vi "PicoScope3000aAdvancedTriggerSettingsV2.vi"(0 "error in":errorcluster, 1 "handle in":i16, 3 "Trigger Conditions":T6 {"Condition Logic" items=["AND", "OR", "XOR"]}, 4 "Trigger Delay":u32, 5 "Auto Trigger (ms)":i32, 6 "Channel A Trigger Properties":T3 {"Direction" items=["Above / Inside", "Below / Outside", "Rising / Enter", "Falling / Exit", "Rising or Falling / Enter or Exit", "Above Lower", "Below Lower", "Rising Lower", "Falling Lower", "Positive Runt", "Negative Runt"]; "Threshold Mode" items=["Level", "Window"]}, 7 "Channel D Trigger Properties":T3 {"Direction" items=["Above / Inside", "Below / Outside", "Rising / Enter", "Falling / Exit", "Rising or Falling / Enter or Exit", "Above Lower", "Below Lower", "Rising Lower", "Falling Lower", "Positive Runt", "Negative Runt"]; "Threshold Mode" items=["Level", "Window"]}, 8 "Channel B Trigger Properties":T3 {"Direction" items=["Above / Inside", "Below / Outside", "Rising / Enter", "Falling / Exit", "Rising or Falling / Enter or Exit", "Above Lower", "Below Lower", "Rising Lower", "Falling Lower", "Positive Runt", "Negative Runt"]; "Threshold Mode" items=["Level", "Window"]}, 10 "Digital Port  0":T2 {"Direction Channel 7" items=["Don't Care", "Low", "High", "Rising", "Falling"]; "Direction Channel 6" items=["Don't Care", "Low", "High", "Rising", "Falling"]; "Direction Channel 5" items=["Don't Care", "Low", "High", "Rising", "Falling"]; "Direction Channel 4" items=["Don't Care", "Low", "High", "Rising", "Falling"]; "Direction Channel 3" items=["Don't Care", "Low", "High", "Rising", "Falling"]; "Direction Channel 2" items=["Don't Care", "Low", "High", "Rising", "Falling"]; "Direction Channel 1" items=["Don't Care", "Low", "High", "Rising", "Falling"]; "Direction Channel 0" items=["Don't Care", "Low", "High", "Rising", "Falling"]}, 11 "Ext. Trigger Properties":T3 {"Direction" items=["Above / Inside", "Below / Outside", "Rising / Enter", "Falling / Exit", "Rising or Falling / Enter or Exit", "Above Lower", "Below Lower", "Rising Lower", "Falling Lower", "Positive Runt", "Negative Runt"]; "Threshold Mode" items=["Level", "Window"]}, 12 "Digital Port  1":T1 {"Direction Channel 15" items=["Don't Care", "Low", "High", "Rising", "Falling"]; "Direction Channel 14" items=["Don't Care", "Low", "High", "Rising", "Falling"]; "Direction Channel 13" items=["Don't Care", "Low", "High", "Rising", "Falling"]; "Direction Channel 12" items=["Don't Care", "Low", "High", "Rising", "Falling"]; "Direction Channel 11" items=["Don't Care", "Low", "High", "Rising", "Falling"]; "Direction Channel 10" items=["Don't Care", "Low", "High", "Rising", "Falling"]; "Direction Channel 9" items=["Don't Care", "Low", "High", "Rising", "Falling"]; "Direction Channel 8" items=["Don't Care", "Low", "High", "Rising", "Falling"]}, 13 "Aux. Trigger Properties":T3 {"Direction" items=["Above / Inside", "Below / Outside", "Rising / Enter", "Falling / Exit", "Rising or Falling / Enter or Exit", "Above Lower", "Below Lower", "Rising Lower", "Falling Lower", "Positive Runt", "Negative Runt"]; "Threshold Mode" items=["Level", "Window"]}, 16 "Channel C Trigger Properties":T3 {"Direction" items=["Above / Inside", "Below / Outside", "Rising / Enter", "Falling / Exit", "Rising or Falling / Enter or Exit", "Above Lower", "Below Lower", "Rising Lower", "Falling Lower", "Positive Runt", "Negative Runt"]; "Threshold Mode" items=["Level", "Window"]}, 18 "Pulse Width Qualifier Conditions":T5 {"Condition Logic" items=["AND", "OR", "XOR"]}, 19 "Pulse Width Qualifier Settings":T4 {"Pulse Width Type" items=["None", "Less Than", "Greater Than", "In Range", "Out of Range"]; "Direction" items=["Rising", "Falling"]}) -> (14 "error out":errorcluster, 15 "handle out":i16)   [LabVIEW 2009]
doc: "This VI is an interface for the advanced trigger features of the oscilloscope (a simple trigger can be set using PicoScope3000aSettings.vi, in which case it is not necessary to use this VI)."
uses:
  ps3000a.dll
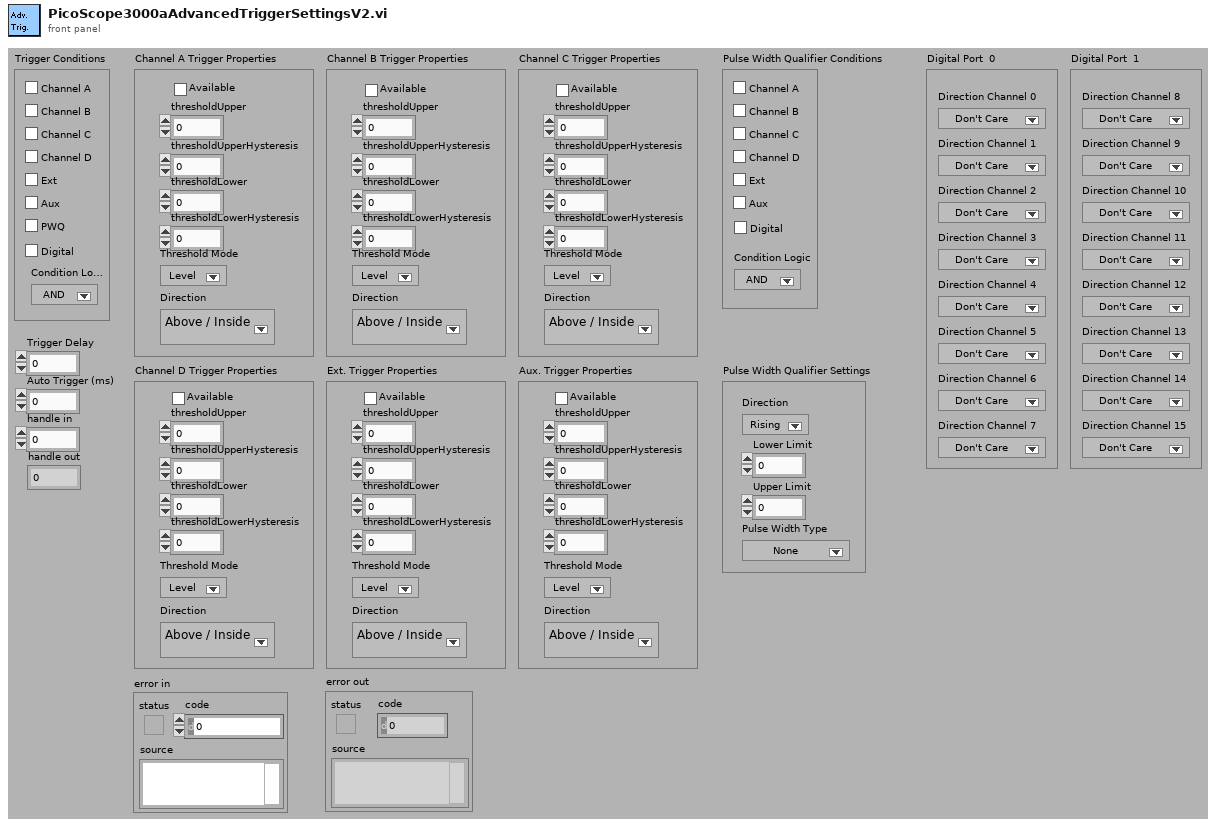
[diagram p1: front panel]
types:
  T1 = cluster{"Direction Channel 8":u16, "Direction Channel 9":u16, "Direction Channel 10":u16, "Direction Channel 11":u16, "Direction Channel 12":u16, "Direction Channel 13":u16, "Direction Channel 14":u16, "Direction Channel 15":u16}
  T2 = cluster{"Direction Channel 0":u16, "Direction Channel 1":u16, "Direction Channel 2":u16, "Direction Channel 3":u16, "Direction Channel 4":u16, "Direction Channel 5":u16, "Direction Channel 6":u16, "Direction Channel 7":u16}
  T3 = cluster{"thresholdUpper":i16, "thresholdUpperHysteresis":u16, "thresholdLower":i16, "thresholdLowerHysteresis":u16, "Threshold Mode":i32, "Direction":i32, "Available":bool}
  T4 = cluster{"Direction":u32, "Lower Limit":u32, "Upper Limit":u32, "Pulse Width Type":u32}
  T5 = cluster{"Channel A":bool, "Channel B":bool, "Channel C":bool, "Channel D":bool, "Aux":bool, "Condition Logic":u16, "Ext":bool, "Digital":bool}
  T6 = cluster{"Channel A":bool, "Channel B":bool, "Channel C":bool, "Channel D":bool, "Aux":bool, "PWQ":bool, "Condition Logic":u16, "Ext":bool, "Digital":bool}
  T7 = cluster{"thresholdUpper":i16, "thresholdUpperHysteresis":u16, "thresholdLower":i16, "thresholdLowerHysteresis":u16, "Threshold Mode":i32, "Direction":i32, "Available":bool}[]
  T8 = cluster{"[0]":u32, "[1]":u32, "[2]":u32, "[3]":u32, "[4]":u32, "[5]":u32, "[6]":u32, "[7]":u32, "[8]":u32}
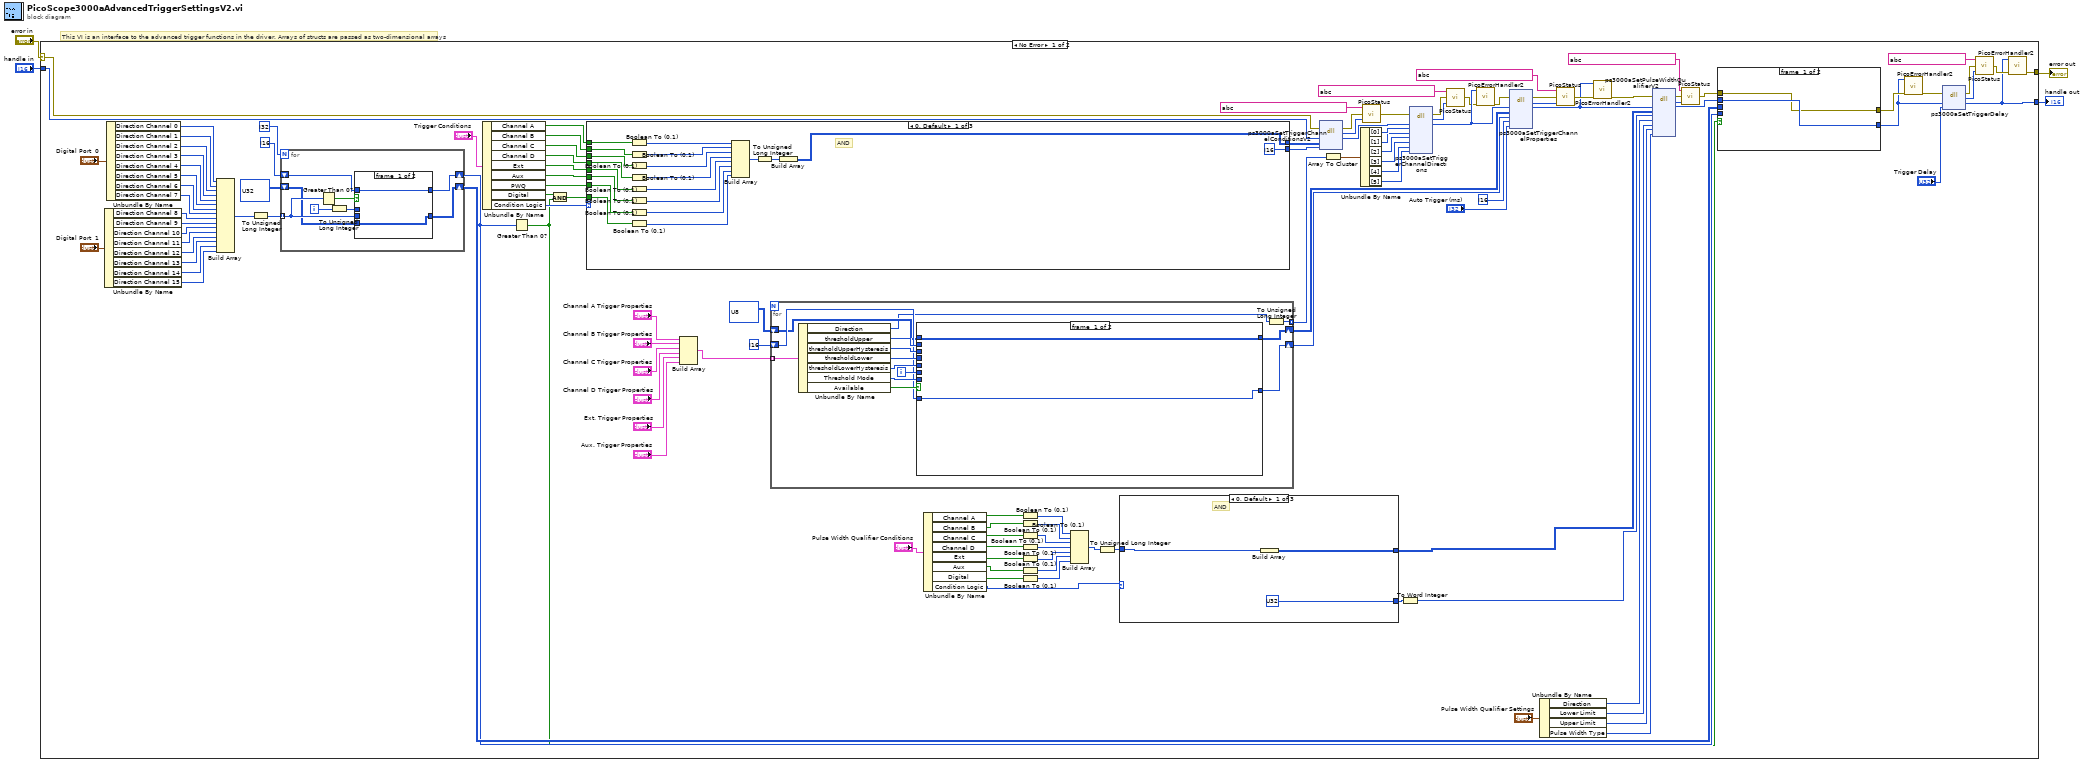
[diagram p0: block diagram]
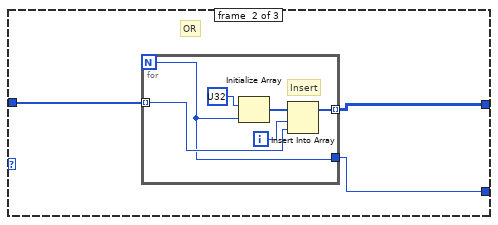
[diagram p2: hidden frame]
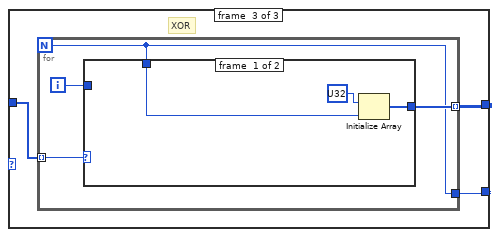
[diagram p3: hidden frame]
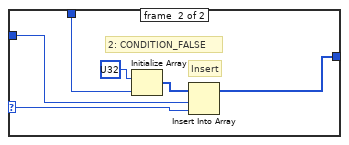
[diagram p4: hidden frame]
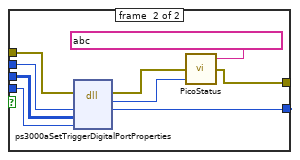
[diagram p5: hidden frame]
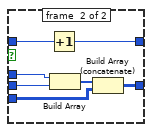
[diagram p6: hidden frame]
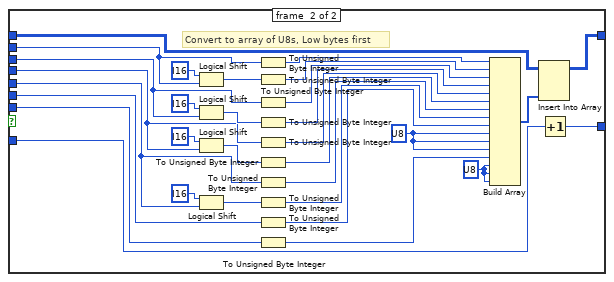
[diagram p7: hidden frame]
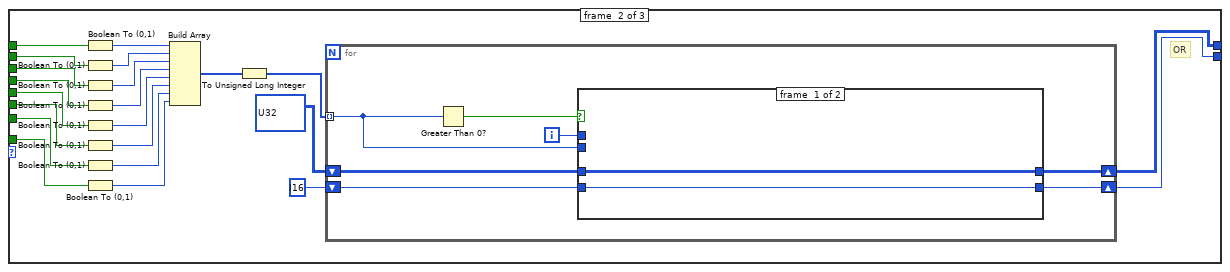
[diagram p8: hidden frame]
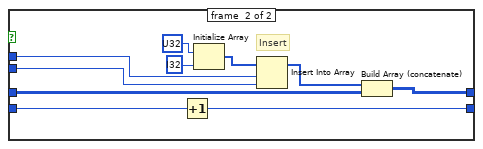
[diagram p9: hidden frame]
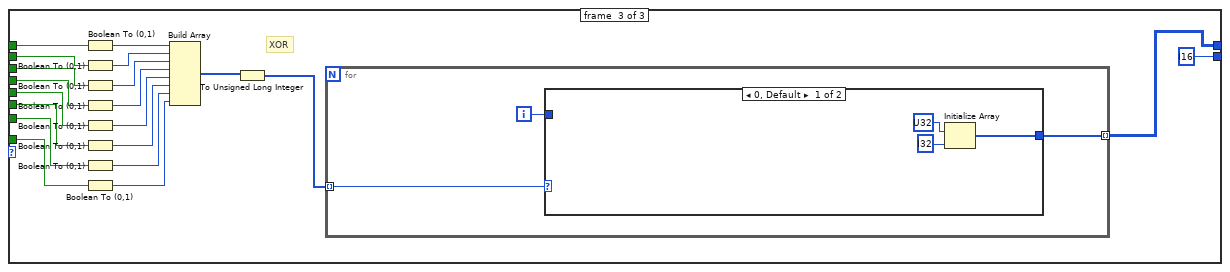
[diagram p10: hidden frame]
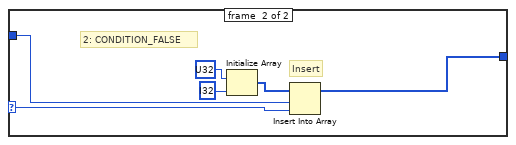
[diagram p11: hidden frame]
diagram:
  # "This VI is an interface to the advanced trigger functions in the driver. Arrays of structs are passed as two-dimensional arrays"
  n1 = case shown="No Error" "error in" {
    selector: "error in" -> [w93 w321]
    tunnel: "handle in" -> [w97 w322]
    tunnel: [w33 w322] -> w2
    tunnel: [w34 w321] -> w1
    frame #0 {
      n2 = Unbundle By Name("Digital Port  1") -> ("Direction Channel 8"=w58:u16, "Direction Channel 9"=w57:u16, "Direction Channel 10"=w56:u16, "Direction Channel 11"=w55:u16, "Direction Channel 12"=w54:u16, "Direction Channel 13"=w53:u16, "Direction Channel 14"=w52:u16, "Direction Channel 15"=w51:u16)
      n3 = Unbundle By Name("Digital Port  0") -> ("Direction Channel 0"=w70:u16, "Direction Channel 1"=w69:u16, "Direction Channel 2"=w68:u16, "Direction Channel 3"=w67:u16, "Direction Channel 4"=w66:u16, "Direction Channel 5"=w65:u16, "Direction Channel 6"=w64:u16, "Direction Channel 7"=w63:u16)
      n4 = Build Array(w70, w69, w68, w67, w66, w65, w64, w63, w58, w57, w56, w55, w54, w53, w52, w51) -> (w25:u16[])
      n5 = To Unsigned Long Integer(number=w25) -> (unsigned 32bit integer=w26:u32[])
      n6 = for {
        N: i32 ? -> [_]
        tunnel: w26 -> [w170] mode=indexing
        shift-right: [w169] -> w46
        shift-left: u32[][] ? -> [w168]
        shift-right: [w167] -> w43
        shift-left: i16 ? -> [w166]
        i -> [w164]
        n7 = Greater Than 0?(x=w170) -> (x > 0?=w171:bool)
        n8 = To Unsigned Long Integer(number=w164) -> (unsigned 32bit integer=w165:u32)
        n9 = case shown="True" w171 {
          tunnel: w165 -> [_ w180]
          tunnel: w170 -> [_ w179]
          tunnel: [w173 w177] -> w169
          tunnel: w168 -> [w173 w176]
          tunnel: [w172 w175] -> w167
          tunnel: w166 -> [w172 w174]
          frame #0 {
          }
          frame #1 {
            n10 = Increment(x=w174) -> (x+1=w175:i16)
            n11 = Build Array(w180, w179) -> (w178:u32[])
            n12 = Build Array (concatenate)(w178, w176) -> (w177:u32[][])
          }
        }
      }
      n13 = Unbundle By Name("Trigger Conditions") -> ("Channel A"=w77:bool, "Channel B"=w76:bool, "Channel C"=w75:bool, "Channel D"=w74:bool, "Ext"=w73:bool, "Aux"=w72:bool, "PWQ"=w71:bool, "Digital"=w45:bool, "Condition Logic"=w78:u16)
      n14 = Greater Than 0?(x=w43) -> (x > 0?=w42:bool)
      n15 = And(x=w45, y=w42) -> (x .and. y?=w44:bool)
      n16 = case shown="0, Default" w78 {
        tunnel: [w247 w262 w301] -> w121
        tunnel: [i16 ? w260 i16 ?] -> w120
        tunnel: w77 -> [w245 w257 w298]
        tunnel: w76 -> [w244 w256 w297]
        tunnel: w75 -> [w243 w255 w296]
        tunnel: w74 -> [w242 w254 w295]
        tunnel: w73 -> [w241 w253 w294]
        tunnel: w72 -> [w240 w252 w293]
        tunnel: w71 -> [w239 w251 w292]
        tunnel: w44 -> [w238 w250 w291]
        frame #0 {
          # "AND"
          n17 = Boolean To (0,1)(Boolean=w245) -> (0, 1=w237:i16)
          n18 = Boolean To (0,1)(Boolean=w244) -> (0, 1=w236:i16)
          n19 = Boolean To (0,1)(Boolean=w243) -> (0, 1=w230:i16)
          n20 = Boolean To (0,1)(Boolean=w242) -> (0, 1=w231:i16)
          n21 = Boolean To (0,1)(Boolean=w241) -> (0, 1=w232:i16)
          n22 = Boolean To (0,1)(Boolean=w240) -> (0, 1=w233:i16)
          n23 = Boolean To (0,1)(Boolean=w239) -> (0, 1=w234:i16)
          n24 = Boolean To (0,1)(Boolean=w238) -> (0, 1=w235:i16)
          n25 = Build Array(w237, w236, w230, w231, w232, w233, w234, w235) -> (w229:i16[])
          n26 = To Unsigned Long Integer(number=w229) -> (unsigned 32bit integer=w228:u32[])
          n27 = Build Array(w228) -> (w247:u32[][])
        }
        frame #1 {
          # "OR"
          n28 = Boolean To (0,1)(Boolean=w257) -> (0, 1=w263:i16)
          n29 = Boolean To (0,1)(Boolean=w256) -> (0, 1=w264:i16)
          n30 = Boolean To (0,1)(Boolean=w255) -> (0, 1=w265:i16)
          n31 = Boolean To (0,1)(Boolean=w254) -> (0, 1=w266:i16)
          n32 = Boolean To (0,1)(Boolean=w253) -> (0, 1=w267:i16)
          n33 = Boolean To (0,1)(Boolean=w252) -> (0, 1=w268:i16)
          n34 = Boolean To (0,1)(Boolean=w251) -> (0, 1=w269:i16)
          n35 = Boolean To (0,1)(Boolean=w250) -> (0, 1=w258:i16)
          n36 = Build Array(w263, w264, w265, w266, w267, w268, w269, w258) -> (w249:i16[])
          n37 = To Unsigned Long Integer(number=w249) -> (unsigned 32bit integer=w248:u32[])
          n38 = for {
            tunnel: w248 -> [w273] mode=indexing
            shift-right: [w272] -> w262
            shift-left: u32[][] ? -> [w276]
            shift-right: [w270] -> w260
            shift-left: i16 ? -> [w271]
            i -> [w275]
            n39 = Greater Than 0?(x=w273) -> (x > 0?=w274:bool)
            n40 = case shown="True" w274 {
              tunnel: w276 -> [w278 w281]
              tunnel: w275 -> [_ w285]
              tunnel: w273 -> [_ w284]
              tunnel: [w278 w283] -> w272
              tunnel: w271 -> [w277 w280]
              tunnel: [w277 w279] -> w270
              frame #0 {
              }
              frame #1 {
                # "Insert"
                n41 = Increment(x=w280) -> (x+1=w279:i16)
                n42 = Initialize Array(u32 ? ("element"), i32 ? ("dimension size")) -> (w286:u32[])
                n43 = Insert Into Array(array=w286, index=w285, new element=w284) -> (w282:u32[])
                n44 = Build Array (concatenate)(w282, w281) -> (w283:u32[][])
              }
            }
          }
        }
        frame #2 {
          # "XOR"
          n45 = Boolean To (0,1)(Boolean=w298) -> (0, 1=w302:i16)
          n46 = Boolean To (0,1)(Boolean=w297) -> (0, 1=w303:i16)
          n47 = Boolean To (0,1)(Boolean=w296) -> (0, 1=w304:i16)
          n48 = Boolean To (0,1)(Boolean=w295) -> (0, 1=w305:i16)
          n49 = Boolean To (0,1)(Boolean=w294) -> (0, 1=w306:i16)
          n50 = Boolean To (0,1)(Boolean=w293) -> (0, 1=w307:i16)
          n51 = Boolean To (0,1)(Boolean=w292) -> (0, 1=w308:i16)
          n52 = Boolean To (0,1)(Boolean=w291) -> (0, 1=w299:i16)
          n53 = Build Array(w302, w303, w304, w305, w306, w307, w308, w299) -> (w290:i16[])
          n54 = To Unsigned Long Integer(number=w290) -> (unsigned 32bit integer=w289:u32[])
          n55 = for {
            tunnel: w289 -> [w309] mode=indexing
            tunnel: [w311] -> w301 mode=indexing
            i -> [w310]
            n56 = case shown="0, Default" w309 {
              selector: w309 -> [_ w316]
              tunnel: [w312 w317] -> w311
              tunnel: w310 -> [_ w315]
              frame #0 {
                n57 = Initialize Array(u32 ? ("element"), i32 ? ("dimension size")) -> (w312:u32[])
              }
              frame #1 {
                # "2: CONDITION_FALSE"
                # "Insert"
                n58 = Initialize Array(u32 ? ("element"), i32 ? ("dimension size")) -> (w318:u32[])
                n59 = Insert Into Array(array=w318, index=w315, new element=w316) -> (w317:u32[])
              }
            }
          }
        }
      }
      n60 = Build Array("Channel A Trigger Properties", "Channel B Trigger Properties", "Channel C Trigger Properties", "Channel D Trigger Properties", "Ext. Trigger Properties", "Aux. Trigger Properties") -> (w118:T7)
      n61 = for {
        tunnel: w118 -> [w189] mode=indexing
        tunnel: [w182] -> w117 mode=indexing
        shift-right: [w186] -> w81
        shift-left: i16 ? -> [w185]
        shift-right: [w183] -> w79
        shift-left: u8[][] ? -> [w184]
        i -> [w187]
        n62 = Unbundle By Name(w189) -> ("Direction"=w181:i32, "thresholdUpper"=w194:i16, "thresholdUpperHysteresis"=w193:u16, "thresholdLower"=w192:i16, "thresholdLowerHysteresis"=w191:u16, "Threshold Mode"=w190:i32, "Available"=w188:bool)
        n63 = case shown="True" w188 {
          tunnel: w194 -> [_ w226]
          tunnel: w193 -> [_ w218]
          tunnel: w192 -> [_ w217]
          tunnel: w191 -> [_ w216]
          tunnel: w190 -> [_ w207]
          tunnel: w187 -> [_ w202]
          tunnel: [w196 w201] -> w186
          tunnel: w185 -> [w196 w200]
          tunnel: [w195 w198] -> w183
          tunnel: w184 -> [w195 w197]
          frame #0 {
          }
          frame #1 {
            w205 = u8 ? ("element")
            w206 = u8 ? ("element")
            # "Convert to array of U8s, Low bytes first"
            n64 = Logical Shift(y=i16 ?, x=w226) -> (x << y=w225:i16)
            n65 = Logical Shift(y=i16 ?, x=w218) -> (x << y=w224:u16)
            n66 = Logical Shift(y=i16 ?, x=w217) -> (x << y=w221:i16)
            n67 = Logical Shift(y=i16 ?, x=w216) -> (x << y=w220:u16)
            n68 = To Unsigned Byte Integer(number=w226) -> (unsigned 8bit integer=w215:u8)
            n69 = To Unsigned Byte Integer(number=w225) -> (unsigned 8bit integer=w214:u8)
            n70 = To Unsigned Byte Integer(number=w218) -> (unsigned 8bit integer=w213:u8)
            n71 = To Unsigned Byte Integer(number=w224) -> (unsigned 8bit integer=w212:u8)
            n72 = To Unsigned Byte Integer(number=w217) -> (unsigned 8bit integer=w211:u8)
            n73 = To Unsigned Byte Integer(number=w221) -> (unsigned 8bit integer=w210:u8)
            n74 = To Unsigned Byte Integer(number=w216) -> (unsigned 8bit integer=w209:u8)
            n75 = To Unsigned Byte Integer(number=w220) -> (unsigned 8bit integer=w208:u8)
            n76 = To Unsigned Byte Integer(number=w202) -> (unsigned 8bit integer=w203:u8)
            n77 = To Unsigned Byte Integer(number=w207) -> (unsigned 8bit integer=w204:u8)
            n78 = Build Array(w215, w214, w213, w212, w211, w210, w209, w208, w203, w206, w206, w206, w204, w205, w205, w205) -> (w199:u8[])
            n79 = Insert Into Array(array=w197, new element=w199) -> (w198:u8[][])  [unwired: 2 in]
            n80 = Increment(x=w200) -> (x+1=w201:i16)
          }
        }
        n81 = To Unsigned Long Integer(number=w181) -> (unsigned 32bit integer=w182:u32)
      }
      n82 = Unbundle By Name("Pulse Width Qualifier Conditions") -> ("Channel A"=w8:bool, "Channel B"=w9:bool, "Channel C"=w10:bool, "Channel D"=w11:bool, "Ext"=w12:bool, "Aux"=w13:bool, "Digital"=w14:bool, "Condition Logic"=w15:u16)
      n83 = Boolean To (0,1)(Boolean=w8) -> (0, 1=w7:i16)
      n84 = Boolean To (0,1)(Boolean=w9) -> (0, 1=w20:i16)
      n85 = Boolean To (0,1)(Boolean=w10) -> (0, 1=w21:i16)
      n86 = Boolean To (0,1)(Boolean=w11) -> (0, 1=w22:i16)
      n87 = Boolean To (0,1)(Boolean=w12) -> (0, 1=w23:i16)
      n88 = Boolean To (0,1)(Boolean=w13) -> (0, 1=w24:i16)
      n89 = Boolean To (0,1)(Boolean=w14) -> (0, 1=w19:i16)
      n90 = Build Array(w7, w20, w21, w22, w23, w24, w19) -> (w18:i16[])
      n91 = To Unsigned Long Integer(number=w18) -> (unsigned 32bit integer=w17:u32[])
      n92 = case shown="0, Default" w15 {
        tunnel: [w127 w130 w139] -> w5
        tunnel: [u32 ? w128 w138] -> w16
        tunnel: w17 -> [w125 w129 w137]
        frame #0 {
          # "AND"
          n93 = Build Array(w125) -> (w127:u32[][])
        }
        frame #1 {
          # "OR"
          n94 = for {
            N -> [w131]
            tunnel: w129 -> [w133] mode=indexing
            tunnel: [w132] -> w130 mode=indexing
            tunnel: [w131] -> w128
            i -> [w134]
            # "Insert"
            n95 = Initialize Array(u32 ? ("element"), w131) -> (w135:u32[])
            n96 = Insert Into Array(array=w135, index=w134, new element=w133) -> (w132:u32[])
          }
        }
        frame #2 {
          # "XOR"
          n97 = for {
            N -> [w140]
            tunnel: w137 -> [w143] mode=indexing
            tunnel: [w141] -> w139 mode=indexing
            tunnel: [w140] -> w138
            i -> [w142]
            n98 = case shown="1" w143 {
              selector: w143 -> [_ w149]
              tunnel: [w145 w150] -> w141
              tunnel: w142 -> [_ w148]
              tunnel: w140 -> [w144 w147]
              frame #0 {
                n99 = Initialize Array(u32 ? ("element"), w144) -> (w145:u32[])
              }
              frame #1 {
                # "2: CONDITION_FALSE"
                # "Insert"
                n100 = Initialize Array(u32 ? ("element"), w147) -> (w151:u32[])
                n101 = Insert Into Array(array=w151, index=w148, new element=w149) -> (w150:u32[])
              }
            }
          }
        }
      }
      n102 = dll-call lib="ps3000a.dll" fn="ps3000aSetTriggerChannelConditionsV2" ("ps3000.dll:_ps3000_open_unit@0")(error in=w93, "handle"=w97, "conditions"=w121, "nConditions"=w120) -> (error out=w95:errorcluster, "PICO_STATUS"=w96:i32, "handle"=w123:i16)  [unwired: 4 in, 1 out]
      n103 = Array To Cluster(array=w117) -> (cluster=w116:T8)
      n104 = Unbundle By Name(w116) -> ("[0]"=w115:u32, "[1]"=w114:u32, "[2]"=w113:u32, "[3]"=w112:u32, "[4]"=w111:u32, "[5]"=w110:u32)
      n105 = call "PicoStatus.vi"("PICO STATUS"=w96, "error in"=w95, "source"=string ?) -> ("error out"=w92:errorcluster)
      n106 = To Word Integer(number=w16) -> (16bit integer=w6:i16)
      n107 = dll-call lib="ps3000a.dll" fn="ps3000aSetTriggerChannelDirections" ("ps3000.dll:_ps3000_open_unit@0")(error in=w92, "handle"=w123, "channelA"=w115, "channelB"=w114, "channelC"=w113, "channelD"=w112, "ext"=w111, "aux"=w110) -> (error out=w90:errorcluster, "PICO_STATUS"=w91:i32, "handle"=w40:i16)  [unwired: 8 in, 1 out]
      n108 = call "PicoStatus.vi"("PICO STATUS"=w91, "error in"=w90, "source"=string ?) -> ("error out"=w39:errorcluster)
      n109 = call "PicoErrorHandler2.vi"("error in (no error)"=w39, "handle In"=w40) -> ("error out"=w41:errorcluster)  [unwired: 9 in]
      n110 = dll-call lib="ps3000a.dll" fn="ps3000aSetTriggerChannelProperties" ("ps3000.dll:_ps3000_open_unit@0")(error in=w41, "handle"=w40, "channelProperties"=w79, "nChannelProperties"=w81, "auxOutputEnable"=i16 ?, "autoTriggerMilliseconds"="Auto Trigger (ms)") -> (error out=w88:errorcluster, "PICO_STATUS"=w89:i32, "handle"=w30:i16)  [unwired: 6 in, 1 out]
      n111 = Unbundle By Name("Pulse Width Qualifier Settings") -> ("Direction"=w106:u32, "Lower Limit"=w105:u32, "Upper Limit"=w104:u32, "Pulse Width Type"=w103:u32)
      n112 = call "PicoStatus.vi"("PICO STATUS"=w89, "error in"=w88, "source"=string ?) -> ("error out"=w31:errorcluster)
      n113 = call "PicoErrorHandler2.vi"("error in (no error)"=w31, "handle In"=w30) -> ("error out"=w32:errorcluster)  [unwired: 9 in]
      n114 = dll-call lib="ps3000a.dll" fn="ps3000aSetPulseWidthQualifierV2" ("ps3000.dll:_ps3000_open_unit@0")(error in=w32, "handle"=w30, "conditions"=w5, "nConditions"=w6, "direction"=w106, "lower"=w105, "upper"=w104, "type"=w103) -> (error out=w37:errorcluster, "PICO_STATUS"=w38:i32, "handle"=w47:i16)  [unwired: 8 in, 1 out]
      n115 = call "PicoStatus.vi"("PICO STATUS"=w38, "error in"=w37, "source"=string ?) -> ("error out"=w48:errorcluster)
      n116 = case shown="True" w42 {
        tunnel: w48 -> [w153 w162]
        tunnel: w47 -> [w154 w161]
        tunnel: [w154 w156] -> w28
        tunnel: w43 -> [_ w157]
        tunnel: w46 -> [_ w158]
        tunnel: [w153 w155] -> w29
        frame #0 {
        }
        frame #1 {
          n117 = dll-call lib="ps3000a.dll" fn="ps3000aSetTriggerDigitalPortProperties"(error in=w162, "handle"=w161, "digitalDirections"=w158, "nDigitalDirections"=w157) -> (error out=w160:errorcluster, "PICO_STATUS"=w159:i32, "handle"=w156:i16)  [unwired: 4 in, 1 out]
          n118 = call "PicoStatus.vi"("PICO STATUS"=w159, "error in"=w160, "source"=string ?) -> ("error out"=w155:errorcluster)
        }
      }
      n119 = call "PicoErrorHandler2.vi"("error in (no error)"=w29, "handle In"=w28) -> ("error out"=w27:errorcluster)  [unwired: 9 in]
      n120 = dll-call lib="ps3000a.dll" fn="ps3000aSetTriggerDelay" ("ps3000.dll:_ps3000_open_unit@0")(error in=w27, "handle"=w28, "delay"="Trigger Delay") -> (error out=w86:errorcluster, "PICO_STATUS"=w87:i32, "handle"=w33:i16)  [unwired: 3 in, 1 out]
      n121 = call "PicoStatus.vi"("PICO STATUS"=w87, "error in"=w86, "source"=string ?) -> ("error out"=w35:errorcluster)
      n122 = call "PicoErrorHandler2.vi"("error in (no error)"=w35, "handle In"=w33) -> ("error out"=w34:errorcluster)  [unwired: 9 in]
    }
    frame #1 {
    }
  }
  "handle out" <- w2
  "error out" <- w1
